vi "Create VIs.vi"(8 "error in":errorcluster, 11 "Runner in":refnum<class "Runner.lvclass">) -> (0 "error out":errorcluster, 3 "Runner out":refnum<class "Runner.lvclass">)   [LabVIEW 2026, in "Runner.lvlib" / "Runner.lvclass"]
doc: "Create VIs. This method must be called after all necessary type definitions have been created."
uses:
  Runner.lvclass
  Runner.lvclass/Runner.ctl
  Interfaces/ILogger/ILogger Messages/Log Msg/Log Msg.lvclass/Log Msg.ctl
  <vilib>/ActorFramework/Message Enqueuer/Message Enqueuer.lvclass/Message Enqueuer.ctl
  <vilib>/ActorFramework/Message Enqueuer/Enqueue.vi
  Interfaces/ILogger/ILogger Messages/Log Msg/Log Msg.lvclass
  <vilib>/ActorFramework/Message Priority Queue/Priority Enqueue.vi
  Interfaces/IFile Manager/IFile Manager.lvclass
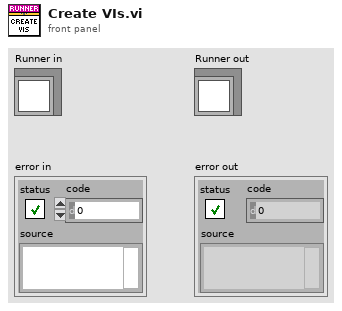
[diagram p1: front panel]
types:
  T1 = typedef "Function--cluster.ctl" = cluster{"name":string, "docstring":string, "input_parameters":T2[], "output_parameters":T2[]}
  T2 = typedef "Parameter--cluster.ctl" = cluster{"name":string, "data_type":string, "container":string, "dimensions":i32, "type_definition":string}
  T3 = typedef "Log Entry--cluster.ctl" = cluster{"Time":timestamp, "Message":string}
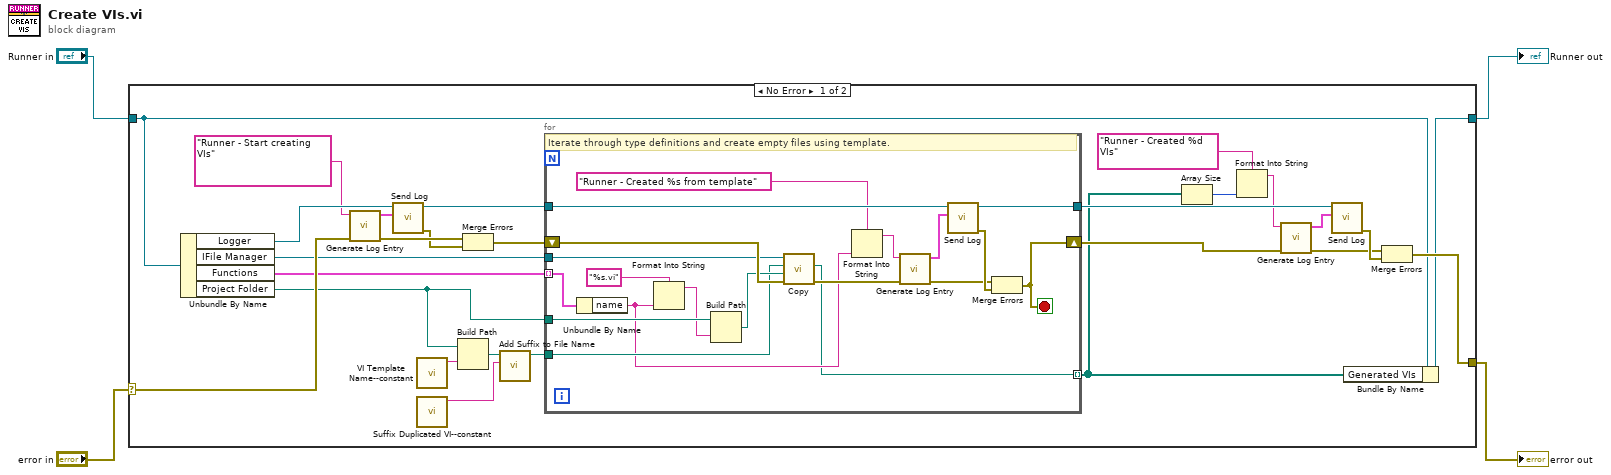
[diagram p0: block diagram]
diagram:
  n1 = case shown="No Error" "error in" {
    selector: "error in" -> [w24 w52]
    tunnel: [w28 w52] -> w3
    tunnel: "Runner in" -> [w23 w51]
    tunnel: [w21 w51] -> w1
    frame No Error {
      n2 = Unbundle By Name(w23) -> ("Logger"=w19:refnum<class "Message Enqueuer.lvclass">, "IFile Manager"=w7:refnum<class "IFile Manager.lvclass">, "Functions"=w22:T1[], "Project Folder"=w20:path)
      n3 = call "Generate Log Entry.vi"("error in"=w24, "Message"="Runner - Start creating VIs") -> ("error out"=w31:errorcluster, "Log Entry"=w17:T3)  [unwired: 8 in]
      n4 = call "Send Log.vi"("Log Entry"=w17, "Message Enqueuer"=w19) -> ("error out"=w29:errorcluster, "Message Enqueuer out"=w18:refnum<class "Message Enqueuer.lvclass">)  [unwired: 8 in]
      n5 = call "VI Template Name--constant.vi"() -> ("VI Template Name"=w5:string)  [unwired: 11 in]
      n6 = call "Suffix Duplicated VI--constant.vi"() -> ("Suffix Duplicated VI"=w8:string)  [unwired: 11 in]
      n7 = Build Path(base path=w20, name or relative path=w5) -> (appended path=w10:path)
      n8 = Merge Errors(w31, w29) -> (w30:errorcluster)
      n9 = call "Add Suffix to File Name.vi"("Suffix"=w8, "File Path in"=w10) -> ("File Path out"=w9:path)  [unwired: 9 in]
      n10 = for {
        tunnel: w22 -> [w45] mode=indexing
        tunnel: w20 -> [w37]
        shift-right: [w49] -> w26
        shift-left: w30 -> [w48]
        tunnel: w9 -> [w34]
        tunnel: w18 -> [w44]
        tunnel: [w40] -> w14
        tunnel: w7 -> [w39]
        tunnel: [w32] -> w6 mode=indexing
        stop <- w49 stop-if-true
        # "Iterate through type definitions and create empty files using template."
        n11 = Unbundle By Name(w45) -> ("name"=w33:string)
        n12 = Format Into String(format string="%s.vi", w33) -> (resulting string=w36:string)  [unwired: 2 in, 1 out]
        n13 = Build Path(base path=w37, name or relative path=w36) -> (appended path=w35:path)
        n14 = call-dynamic "Copy.vi"("error in"=w48, "Target Folder"=w35, "Source File"=w34, "IFile Manager in"=w39) -> ("error out"=w47:errorcluster, "New Path"=w32:path)  [unwired: 5 in, 1 out]
        n15 = Format Into String(format string="Runner - Created %s from template", w33) -> (resulting string=w42:string)  [unwired: 2 in, 1 out]
        n16 = call "Generate Log Entry.vi"("error in"=w47, "Message"=w42) -> ("error out"=w46:errorcluster, "Log Entry"=w41:T3)  [unwired: 8 in]
        n17 = call "Send Log.vi"("Log Entry"=w41, "Message Enqueuer"=w44) -> ("error out"=w50:errorcluster, "Message Enqueuer out"=w40:refnum<class "Message Enqueuer.lvclass">)  [unwired: 8 in]
        n18 = Merge Errors(w46, w50) -> (w49:errorcluster)
      }
      n19 = Array Size(array=w6) -> (size(s)=w12:i32)
      n20 = Format Into String(format string="Runner - Created %d VIs" ("Message"), w12) -> (resulting string=w11:string)  [unwired: 2 in, 1 out]
      n21 = call "Generate Log Entry.vi"("error in"=w26, "Message"=w11) -> ("error out"=w25:errorcluster, "Log Entry"=w15:T3)  [unwired: 8 in]
      n22 = call "Send Log.vi"("Log Entry"=w15, "Message Enqueuer"=w14) -> ("error out"=w27:errorcluster)  [unwired: 8 in, 1 out]
      n23 = Bundle By Name(cluster=w23, "Generated VIs"=w6) -> (w21:refnum<class "Runner.lvclass">)
      n24 = Merge Errors(w25, w27) -> (w28:errorcluster)
    }
    frame Error {
      # "Pass error"
    }
  }
  "error out" <- w3
  "Runner out" <- w1
